vi "Execute.vi"(5 "Username":string, 6 "Password":string, 7 "Address":string, 8 "Error In":errorcluster) -> (0 "Error Out":errorcluster)   [LabVIEW 2018, in "Tests.lvlib" / "Channel.lvlib"]
uses:
  Channel.lvlib
  <vilib>/addons/_JKI Toolkits/Caraya/classes/Test/Test.lvclass
  <vilib>/addons/_JKI Toolkits/Caraya/classes/Assert/Assert.lvclass
  src/Toolkit/Channel/Channel.lvclass
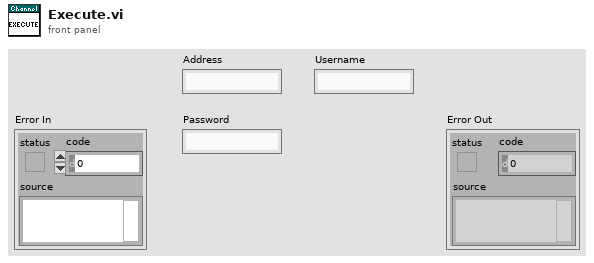
[diagram p1: front panel]
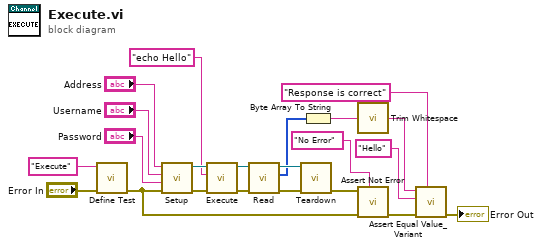
[diagram p0: block diagram]
diagram:
  n1 = call <vilib>:"Define Test.vi"("error in (no error)"="Error In", "Label (VI Title)"="Execute") -> ("error out"=w19:errorcluster)  [unwired: 9 in]
  n2 = call "Setup.vi"("Error In"=w19, "Password"="Password", "Username"="Username", "Address"="Address") -> ("Error Out"=w12:errorcluster, "Channel"=w13:refnum<class "Channel.lvclass">)  [unwired: 6 in]
  n3 = call "Execute.vi"("Error In"=w12, "Command"="echo Hello", "Channel In"=w13) -> ("Error Out"=w9:errorcluster, "Channel Out"=w10:refnum<class "Channel.lvclass">)  [unwired: 7 in]
  n4 = call "Read.vi"("Error In"=w9, "Channel In"=w10) -> ("Error Out"=w8:errorcluster, "Data"=w5:u8[], "Channel Out"=w7:refnum<class "Channel.lvclass">)  [unwired: 7 in]
  n5 = call "Teardown.vi"("Error In"=w8, "Channel"=w7) -> ("Error Out"=w15:errorcluster)  [unwired: 9 in]
  n6 = Byte Array To String(unsigned byte array=w5) -> (string=w2:string)
  n7 = call <vilib>:"Trim Whitespace.vi"("string"=w2) -> ("trimmed string"=w1:string)  [unwired: 1 in]
  n8 = call <vilib>:"Assert Not Error.vi"("Label"="No Error", "error in (no error)"=w19, "Not Error?"=w15) -> ("error out"=w14:errorcluster)  [unwired: 8 in]
  n9 = call <vilib>:"Assert Equal Value_Variant.vi"("Label"="Response is correct", "error in (no error)"=w14, "Y"="Hello" ("string"), "X"=w1) -> ("error out"=→"Error Out":errorcluster)  [unwired: 7 in]
